vi "VIH - CHM Project - Write HHP File - Window Properties.vi"(6 "Default Topic":string, 7 "Window Title":string, 8 "error in":errorcluster, 9 "Index Filename":string, 10 "TOC Filename":string, 11 "queue":T1) -> (0 "error out":errorcluster, 3 "dup queue":T1)   [LabVIEW 2014]
doc: "::: VI Helpeks :::\nCopyright (c) 2000-2026 Konstantin Shifershteyn. All rights reserved."
uses:
  VIH - CHM Project - HHP Support - Queue Refnum.ctl
  VIH - CHM Project - HHP Support - Config Data Cluster.ctl
panel:
  # "VI Helpeks\nCopyright (c) 2012-2026 Konstantin Shifershteyn"
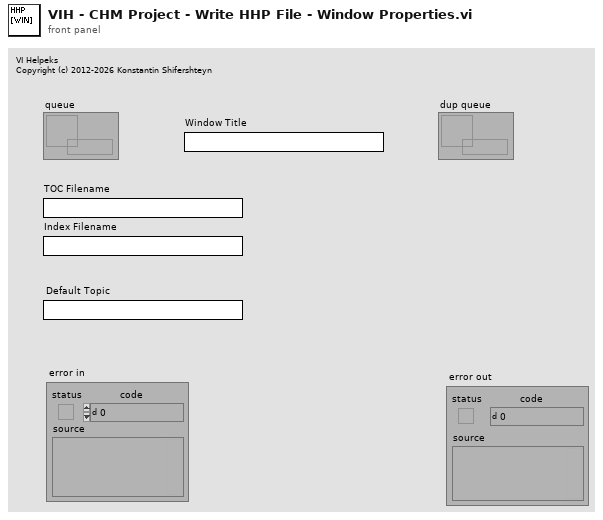
[diagram p1: front panel]
types:
  T1 = typedef "VIH - CHM Project - HHP Support - Queue Refnum.ctl" = refnum<queue>
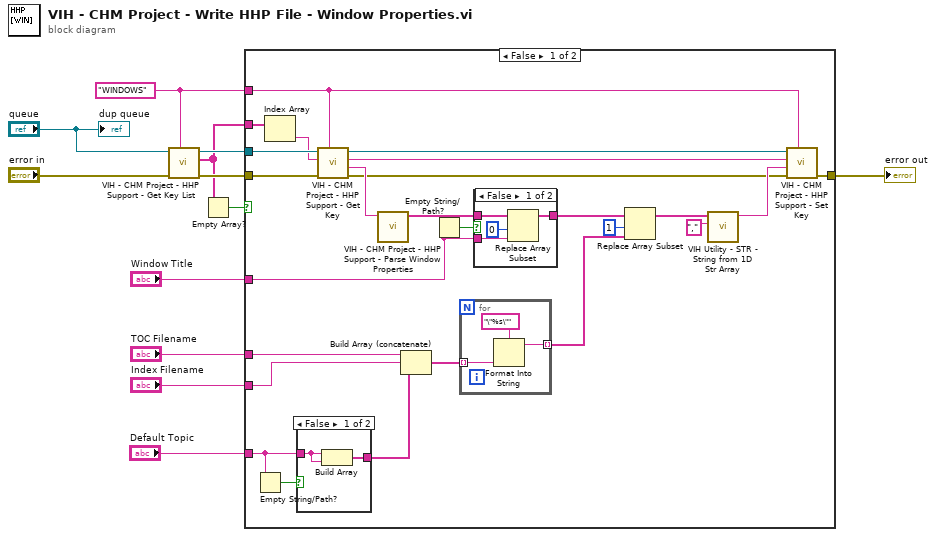
[diagram p0: block diagram]
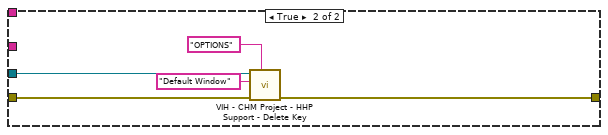
[diagram p4: hidden frame]
diagram:
  w10 = "WINDOWS" ("Section")
  n1 = call "VIH - CHM Project - HHP Support - Get Key List.vi"("Section"=w10, "error in"="error in", "queue"="queue") -> ("error out"=w11:errorcluster, "Keys"=w6:string[], "dup queue"=w12:T1)  [unwired: 6 in]
  n2 = Empty Array?(array=w6) -> (empty?=w5:bool)
  n3 = case shown="False" w5 {
    tunnel: w12 -> [w37 w51]
    tunnel: w11 -> [w35 w52]
    tunnel: w10 -> [w32 _]
    tunnel: [w26 w50] -> w7
    tunnel: w6 -> [w25 _]
    tunnel: "Window Title" -> [w16 _]
    tunnel: "TOC Filename" -> [w21 _]
    tunnel: "Index Filename" -> [w20 _]
    tunnel: "Default Topic" -> [w14 _]
    frame False {
      n4 = Empty String/Path?(string/path=w14) -> (empty?=w15:bool)
      n5 = Index Array(array=w25) -> (element=w36:string)  [unwired: 1 in]
      n6 = case shown="False" w15 {
        tunnel: w14 -> [w39 _]
        tunnel: [w38 _] -> w13
        frame False {
          n7 = Build Array(w39, w39) -> (w38:string[])
        }
        frame True {
        }
      }
      n8 = call "VIH - CHM Project - HHP Support - Get Key.vi"("Section"=w32, "error in"=w35, "Key"=w36, "queue"=w37) -> ("error out"=w27:errorcluster, "Value"=w34:string, "dup Key"=w31:string, "dup queue"=w33:T1)  [unwired: 4 in]
      n9 = call "VIH - CHM Project - HHP Support - Parse Window Properties.vi"("Window property"=w34) -> ("Properties"=w19:string[])  [unwired: 10 in]
      n10 = Build Array (concatenate)(w21, w20, w13) -> (w22:string[])
      n11 = Empty String/Path?(string/path=w16) -> (empty?=w17:bool)
      n12 = for {
        tunnel: [w46] -> w24 mode=indexing
        tunnel: w22 -> [w45] mode=indexing
        n13 = Format Into String(format string="\"%s\"", w45) -> (resulting string=w46:string)  [unwired: 2 in, 1 out]
      }
      n14 = case shown="False" w17 {
        tunnel: w19 -> [w43 w44]
        tunnel: [w42 w44] -> w18
        tunnel: w16 -> [w41 _]
        frame False {
          n15 = Replace Array Subset(array=w43, new element=w41, index=0) -> (w42:string[])
        }
        frame True {
        }
      }
      n16 = Replace Array Subset(array=w18, new element=w24, index=1) -> (w30:string[])
      n17 = call "VIH Utility - STR - String from 1D Str Array.vi"("delimiter ('\\n')"="," ("delimiter ('\\n')"), "Array in"=w30) -> ("String out"=w28:string)  [unwired: 5 in]
      n18 = call "VIH - CHM Project - HHP Support - Set Key.vi"("Section"=w32, "error in"=w27, "Value"=w28, "Key"=w31, "queue"=w33) -> ("error out"=w26:errorcluster)  [unwired: 5 in, 1 out]
    }
    frame True {
      n19 = call "VIH - CHM Project - HHP Support - Delete Key.vi"("Section"="OPTIONS", "error in"=w52, "Key"="Default Window", "queue"=w51) -> ("error out"=w50:errorcluster)  [unwired: 6 in, 1 out]
    }
  }
  "error out" <- w7
  "dup queue" <- "queue"
